vi "Read U8 FIFO.vi"(8 "error in (no error)":errorcluster, 9 "Timeout (ms)":i32, 10 "Data in":u8[](array[numeric]), 11 "CIFFIFO in":refnum<class "CIF_Iceoryx_PCAP_Universal.lvclass">) -> (0 "error out":errorcluster, 1 "timed out?":bool, 2 "Data out":u8[](array[numeric]), 3 "CIFFIFO out":refnum<class "CIF_Iceoryx_PCAP_Universal.lvclass">, 4 "Header":T1)   [LabVIEW 2021, in "CIF_Iceoryx_PCAP_Universal.lvclass"]
uses:
  CIF_Iceoryx_PCAP_Universal.lvclass
  ChannelCommon/typedef/FIFO Header.ctl
  D:/dev/Packages/CIF_Channels_Core/src/CIFChannels/CIFChannels.lvclass
  CIFChannels/CIFChannels.lvclass/CIFChannels.ctl
  CIF_Iceoryx_PCAP_Universal.lvclass/CIF_Iceoryx_PCAP_Universal.ctl
  <vilib>/CIF Foundation/CIF Utilities/Statistics/I64/Stats_I64_CIF_U.lvclass/Stats_I64_CIF_U.ctl
  CIFChannels/Accessors/Read FIFO Payload Length.vi
  CIFChannels/Accessors/Read FIFO Header.vi
  Accessors/Read CIF Subscriber Refnum.vi
  <vilib>/CIF Foundation/CIF Iceoryx/PubSub/CIF pcap/CIF Receive.vi
  ChannelCommon/Utilities/Remove Header Bytes.vi
  CIFChannels/Accessors/Write FIFO Header.vi
  CIFChannels/Utilities/Update Channel Benchmark.vi
  SubVIs/Core Read U8 FIFO.vi/e703c505-0034-46a9-8989-21c0de27793f.vi
  SubVIs/Core Read U8 FIFO.vi/768488f4-e6df-4560-a449-a64b33b49031.vi
  CIFChannels/Accessors/Read Channel State.vi
  CIFChannels/Accessors/Read Direction.vi
  <vilib>/CIF Foundation/CIF Iceoryx/SubVIs/Get Path.vi
  <vilib>/CIF Foundation/CIF Iceoryx/SubVIs/Convert Error.vi
  <vilib>/CIF Foundation/CIF Iceoryx/Refnum/CIF Subscriber from Refnum.vi
  <vilib>/CIF Foundation/CIF Utilities/Statistics/I64/X1 minus X0.vi
  <vilib>/CIF Foundation/CIF Utilities/Time/System Time/Get System Time.vi
  <vilib>/CIF Foundation/CIF Utilities/Statistics/I64/X1 minus X0.vi/dfabcf33-0dbc-4041-80a5-3dc0c86d2989.vi
  <vilib>/CIF Foundation/CIF Utilities/Statistics/I64/X1 minus X0.vi/dfabcf33-0dbc-4041-80a5-3dc0c86d2989.vi/9eb60a9a-770f-4d2d-8b3f-8465c267ecc9.vi
  <vilib>/CIF Foundation/CIF Iceoryx/SubVIs/Convert Error Core.vi
  ChannelCommon/ChannelCommon.lvlib
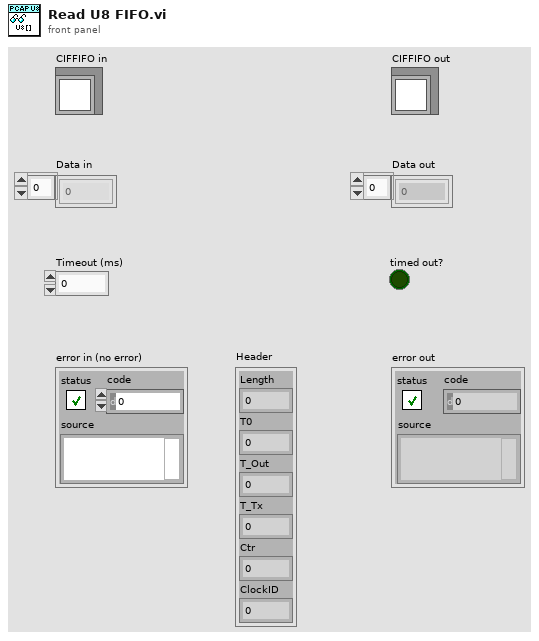
[diagram p1: front panel]
types:
  T1 = typedef "ChannelCommon.lvlib/FIFO Header.ctl" = cluster{"Length":u64, "T0":i64, "T_Out":i64, "T_Tx":i64, "Ctr":u64, "ClockID":u8}
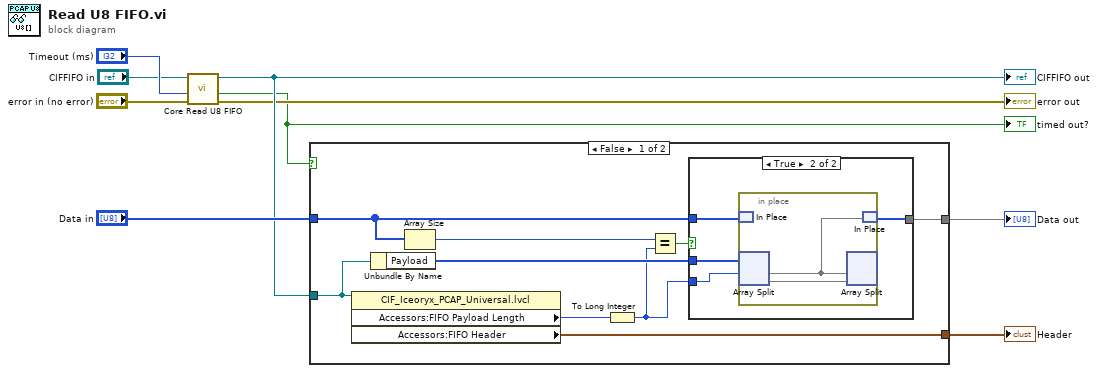
[diagram p0: block diagram]
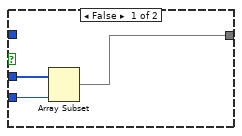
[diagram p2: hidden frame]
diagram:
  n1 = call "Core Read U8 FIFO.vi"("error in (no error)"="error in (no error)", "Timeout (ms)"="Timeout (ms)", "CIFFIFO in"="CIFFIFO in") -> ("error out"=→"error out":errorcluster, "timed out?"=w1:bool, "CIFFIFO out"=w3:refnum<class "CIF_Iceoryx_PCAP_Universal.lvclass">)  [unwired: 6 in]
  "timed out?" <- w1
  "CIFFIFO out" <- w3
  n2 = case shown="False" w1 {
    tunnel: w3 -> [w18 _]
    tunnel: [w16 w28] -> w5
    tunnel: [w15 _] -> w6
    tunnel: "Data in" -> [w12 w28]
    frame False {
      n3 = property class="CIF_Iceoryx_PCAP_Universal.lvcl"(reference=w18) -> ("Accessors:FIFO Payload Length"=w10:u64, "Accessors:FIFO Header"=w15:T1)  [unwired: 1 in, 2 out]
      n4 = Unbundle By Name(w18) -> ("Payload"=w17:u8[])
      n5 = Array Size(array=w12) -> (size(s)=w14:i32)
      n6 = To Long Integer(number=w10) -> (32bit integer=w13:i32)
      n7 = Equal?(x=w14, y=w13) -> (x = y?=w11:bool)
      n8 = case shown="True" w11 {
        tunnel: w17 -> [w21 w24]
        tunnel: [w19 w22] -> w16
        tunnel: w13 -> [w20 w23]
        tunnel: w12 -> [_ w25]
        frame False {
          n9 = Array Subset(array=w21, length=w20) -> (w19:u8[])  [unwired: 1 in]
        }
        frame True {
          n10 = in-place {
            n11 = in-place-match #1(w25) -> ()  [unwired: 1 out]
            n12 = in-place-split #2(w24, w23) -> (w26:u8[], w27:u8[])
            n13 = in-place-split #2(w26, w27) -> ()  [unwired: 2 out]
            n14 = in-place-match #1(w26) -> (w22:u8[])
          }
        }
      }
    }
    frame True {
    }
  }
  "Header" <- w6
  "Data out" <- w5
